vi "Launch System uServices.vi"(8 "error in (no error)":errorcluster, 11 "Guardian in":refnum<class "Guardian.lvclass">) -> (0 "error out":errorcluster, 3 "Guardian out":refnum<class "Guardian.lvclass">)   [LabVIEW 2020, in "TALOS.lvlib" / "Guardian.lvlib" / "Guardian.lvclass"]
uses:
  Guardian.lvclass
  Guardian.lvclass/Guardian.ctl
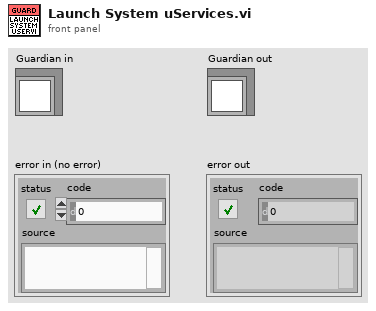
[diagram p1: front panel]
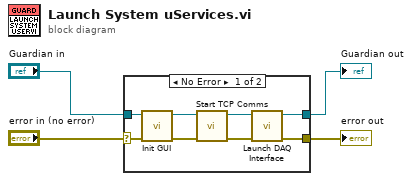
[diagram p0: block diagram]
diagram:
  n1 = case shown="No Error" "error in (no error)" {
    selector: "error in (no error)" -> [w12 w14]
    tunnel: "Guardian in" -> [w11 w13]
    tunnel: [w5 w14] -> w2
    tunnel: [w6 w13] -> w1
    frame No Error {
      n2 = call "Init GUI.vi"("error in (no error)"=w12, "Guardian in"=w11) -> ("error out"=w9:errorcluster, "Guardian out"=w8:refnum<class "Guardian.lvclass">)  [unwired: 8 in]
      n3 = call "Start TCP Comms.vi"("error in (no error)"=w9, "Guardian in"=w8) -> ("error out"=w10:errorcluster, "Guardian out"=w7:refnum<class "Guardian.lvclass">)  [unwired: 8 in]
      n4 = call "Launch DAQ Interface.vi"("error in (no error)"=w10, "Guardian in"=w7) -> ("error out"=w5:errorcluster, "Guardian out"=w6:refnum<class "Guardian.lvclass">)  [unwired: 8 in]
    }
    frame Error {
    }
  }
  "error out" <- w2
  "Guardian out" <- w1
